vi "VIH HelpGen - Write HTML File - External.vi"(8 "error in":errorcluster, 9 "Destination Path":path, 10 "Source Path":path, 11 "Project Tree":T1) -> (0 "error out":errorcluster, 3 "dup Project Tree":T1)   [LabVIEW 2014]
doc: "::: VI Helpeks :::\nCopyright (c) 2000-2026 Konstantin Shifershteyn. All rights reserved."
uses:
  _VIH Project Manager.llb/VIH Project Tree Typedef - Tree Refnum.ctl
panel:
  # "VI Helpeks\nCopyright (c) 2012-2026 Konstantin Shifershteyn"
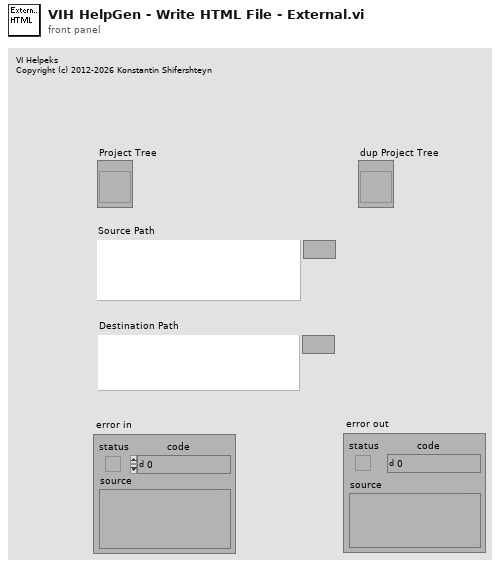
[diagram p1: front panel]
types:
  T1 = typedef "VIH Project Tree Typedef - Tree Refnum.ctl" = refnum<vi>
  T2 = typedef "VIH HelpGen Typedef - Cluster - File Rule.ctl" = cluster{"OutName":string, "BuildHelp":T3, "Source Paths":T4, "Target Paths":T5, "DscrMode":T6, "Description":string, "Control Rules":T7[], "Flags":T9, "Ctl_DscrMode":T6, "Ctl_ClustMembers":T3, "Ctl_EnumValues":T3, "MenuItemIcons":T3, "%Comments":string, "DetailsMode":T6, "DetailsText":string, "ProductInfoMode":T3, "ProductInfoText":string}
  T3 = typedef "VIH HelpGen Typedef - Enum - Default,Enable,Disable.ctl" = enum16{"Default", "Enable", "Disable"}
  T4 = typedef "VIH HelpGen Typedef - Cluster - File Rule - Source Paths.ctl" = cluster{"CSS Files":path[], "JS Files":path[], "Html Template":path}
  T5 = typedef "VIH HelpGen Typedef - Cluster - File Rule - Target Paths.ctl" = cluster{"HTML Dir":path, "Image Dir":path, "CSS Dir":path, "JS Dir":path}
  T6 = typedef "VIH HelpGen Typedef - Enum - Description Mode.ctl" = enum16{"Default", "Description", "Description1", "Description2", "Custom", "None"}
  T7 = typedef "VIH HelpGen Typedef - Cluster - Control Rule.ctl" = cluster{"CtrlID":string, "CustomRule":bool, "DscrMode":T6, "Description":string, "ClusterMembers":T3, "EnumValues":T3, "EnumValDscr":T8[], "CustomName":string}
  T8 = typedef "VIH HelpGen Typedef - Cluster - Enum Value Info.ctl" = cluster{"Value":ext, "String":string, "Description":string}
  T9 = typedef "VIH HelpGen Typedef - Cluster - Group Rule - Flags.ctl" = cluster{"Override CSS Files":bool, "Override JS Files":bool, "Override Ctl Rules":bool}
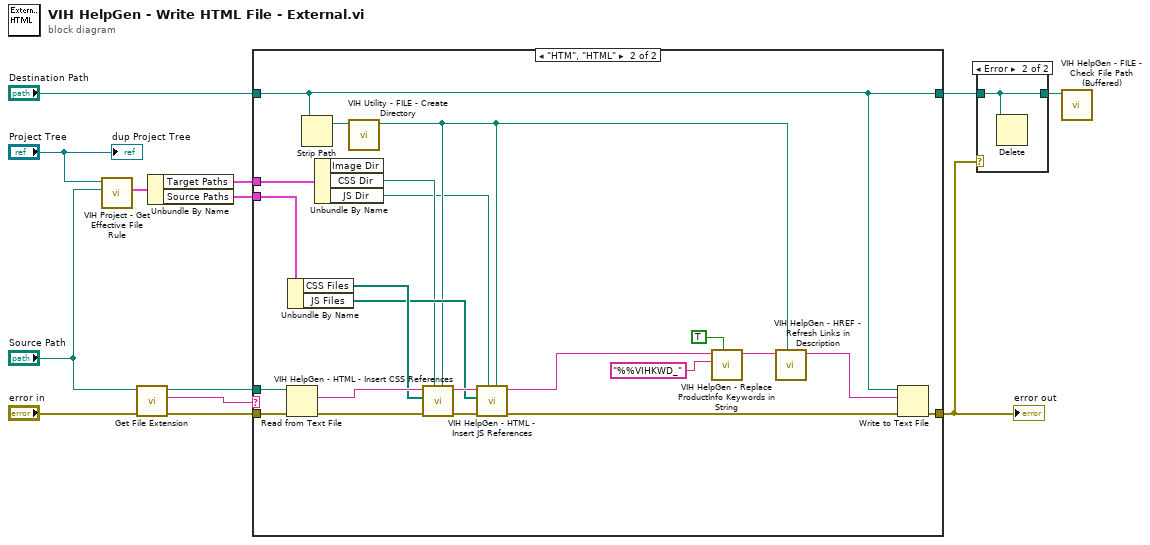
[diagram p0: block diagram]
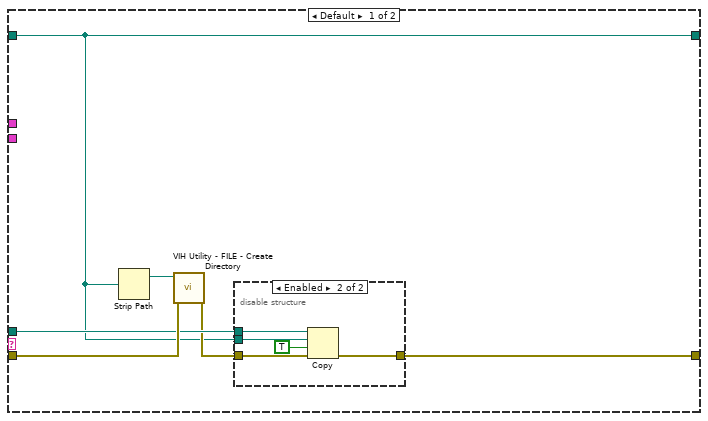
[diagram p3: hidden frame]
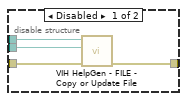
[diagram p4: hidden frame]
diagram:
  n1 = call "VIH Project - Get Effective File Rule.vi"("File Path"="Source Path", "Project Tree"="Project Tree") -> ("Effective File Rule"=w1:T2)  [unwired: 6 in, 3 out]
  n2 = call <vilib>:"Get File Extension.vi"("error in (no error)"="error in", "file"="Source Path") -> ("error out"=w6:errorcluster, "lowercase file extension"=w5:string, "dup file"=w7:path)  [unwired: 6 in, 1 out]
  n3 = Unbundle By Name(w1) -> ("Target Paths"=w13:T5, "Source Paths"=w11:T4)
  n4 = case shown="\"HTM\", \"HTML\"" w5 {
    tunnel: [w15 w50] -> w4
    tunnel: w13 -> [_ w49]
    tunnel: w11 -> [_ w47]
    tunnel: "Destination Path" -> [w14 w34]
    tunnel: w7 -> [w17 w38]
    tunnel: w6 -> [w18 w37]
    tunnel: [w14 w34] -> w3
    frame Default {
      n5 = Strip Path(path=w14) -> (stripped path=w19:path)  [unwired: 1 out]
      n6 = call "VIH Utility - FILE - Create Directory.vi"("error in"=w18, "directory path"=w19) -> ("error out"=w16:errorcluster)  [unwired: 5 in, 2 out]
      n7 = disable-structure shown="Enabled" {
        disable-tunnel: w17 -> [w23 w26]
        disable-tunnel: w16 -> [w22 w27]
        disable-tunnel: [w21 w24] -> w15
        disable-tunnel: w14 -> [w20 w25]
        frame Disabled {
          n8 = call "VIH HelpGen - FILE - Copy or Update File.vi"("error in"=w22, "Target Path"=w20, "Source Path"=w23) -> ("error out"=w21:errorcluster)  [unwired: 7 in, 1 out]
        }
        frame Enabled {
          n9 = Copy(8:w27, 9:TRUE, 10:w25, 11:w26) -> (0:w24:errorcluster)  [unwired: 1 in, 2 out]
        }
      }
    }
    frame "HTM", "HTML" {
      n10 = Read from Text File(file (use dialog)=w38, error in=w37) -> (text=w42:string, error out=w44:errorcluster)  [unwired: 2 in, 2 out]
      n11 = Unbundle By Name(w47) -> ("CSS Files"=w41:path[], "JS Files"=w40:path[])
      n12 = Strip Path(path=w34) -> (stripped path=w48:path)  [unwired: 1 out]
      n13 = Unbundle By Name(w49) -> ("CSS Dir"=w36:path, "JS Dir"=w35:path)  [unwired: 1 out]
      n14 = call "VIH Utility - FILE - Create Directory.vi"("directory path"=w48) -> ("directory path out"=w39:path)  [unwired: 6 in, 2 out]
      n15 = call "VIH HelpGen - HTML - Insert CSS References.vi"("HTML Folder"=w39, "CSS Folder"=w36, "error in"=w44, "CSS files"=w41, "HTML in"=w42) -> ("error out"=w46:errorcluster, "HTML out"=w45:string)  [unwired: 5 in]
      n16 = call "VIH HelpGen - HTML - Insert JS References.vi"("HTML Folder"=w39, "JSS Folder"=w35, "error in"=w46, "JS files"=w40, "HTML in"=w45) -> ("error out"=w43:errorcluster, "HTML out"=w30:string)  [unwired: 5 in]
      n17 = call "VIH HelpGen - Replace ProductInfo Keywords in String.vi"("Coded to HTML (F)"=TRUE, "PINF Prefix"="%%VIHKWD_", "String in"=w30) -> ("String out"=w31:string)  [unwired: 8 in]
      n18 = call "VIH HelpGen - HREF - Refresh Links in Description.vi"("HTML Folder"=w39, "Description in"=w31) -> ("Description out"=w29:string)  [unwired: 9 in]
      n19 = Write to Text File(file (use dialog)=w34, text=w29, error in=w43) -> (error out=w50:errorcluster)  [unwired: 1 in, 2 out]
    }
  }
  "error out" <- w4
  n20 = case shown="Error" w4 {
    tunnel: w3 -> [w51 w52]
    tunnel: [w51 w52] -> w2
    frame No Error {
    }
    frame Error {
      n21 = Delete(path (use dialog)=w52) -> ()  [unwired: 4 in, 3 out]
    }
  }
  n22 = call "VIH HelpGen - FILE - Check File Path (Buffered).vi"("File Path"=w2) -> ()  [unwired: 9 in, 2 out]
  "dup Project Tree" <- "Project Tree"
